vi "Stop Periodic Enqueue Message.vi"(6 "Close Helper Loop (F)":bool, 8 "error in":errorcluster, 11 "Helper Loop":refnum<class "Helper Loop DQMH.lvclass">) -> (0 "error out":errorcluster)   [LabVIEW 2026, in "Helper Loop DQMH.lvclass"]
doc: "周期的処理を終了します。\nClose Helper LoopをTrueにした場合、ヘルパーループを終了し、ユーザーイベントを破棄します。\nClose Helper LoopをFalseにした場合、ヘルパーループを終了させずにヘルパーループを待機状態にします。"
uses:
  Helper Loop DQMH.lvclass
  Helper Loop DQMH.lvclass/Helper Loop DQMH.ctl
  OneDrive/HP/Local/DQMH Helper/Helper Loop/Sub/Helper Loop Map FGV Action.ctl
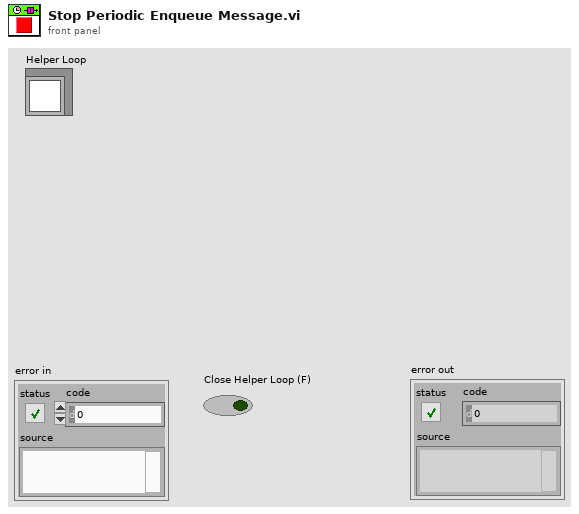
[diagram p1: front panel]
types:
  T1 = typedef "Helper Loop DQMH.lvclass/Helper Loop Map FGV Action.ctl" = enum16{"Get Pausing Helper Loop", "Register Active Helper Loop", "Pause Helper Loop", "Close Helper Loop", "Get All Helper Loops"}
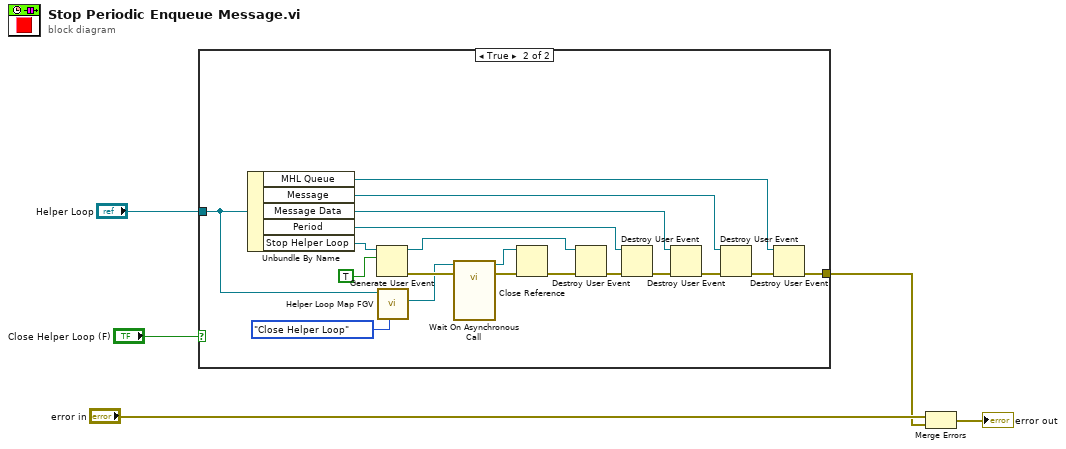
[diagram p0: block diagram]
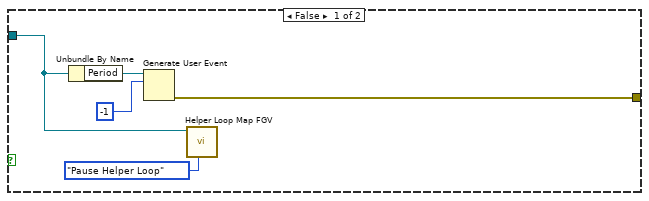
[diagram p2: hidden frame]
diagram:
  n1 = case shown="True" "Close Helper Loop (F)" {
    tunnel: "Helper Loop" -> [w6 w26]
    tunnel: [w8 w18] -> w2
    frame False {
      n2 = Unbundle By Name(w6) -> ("Period"=w10:refnum<user-event>)
      n3 = Generate User Event(user event=w10, event data cluster=-1 ("event data")) -> (error out=w8:errorcluster)  [unwired: 2 in, 1 out]
      n4 = call "Helper Loop Map FGV.vi"("Action"=Helper_Loop_Map_FGV_Action."Pause Helper Loop", "Helper Loop In"=w6) -> ()  [unwired: 6 in, 4 out]
    }
    frame True {
      n5 = Unbundle By Name(w26) -> ("MHL Queue"=w11:refnum<user-event>, "Message"=w12:refnum<user-event>, "Message Data"=w13:refnum<user-event>, "Period"=w14:refnum<user-event>, "Stop Helper Loop"=w29:refnum<user-event>)
      n6 = Generate User Event(user event=w29, event data cluster=TRUE ("event data")) -> (user event out=w20:refnum<user-event>, error out=w27:errorcluster)  [unwired: 2 in]
      n7 = call "Helper Loop Map FGV.vi"("Action"=Helper_Loop_Map_FGV_Action."Close Helper Loop", "Helper Loop In"=w26) -> ("Helper Loop VI Reference Out"=w24:refnum<vi>)  [unwired: 6 in, 3 out]
      n8 = call-by-ref "Wait On Asynchronous Call"(reference=w24, error in=w27) -> (reference out=w22:refnum<vi>, error out=w23:errorcluster)  [unwired: 11 in, 1 out]
      n9 = Close Reference(reference=w22, error in (no error)=w23) -> (error out=w21:errorcluster)
      n10 = Destroy User Event(user event=w20, error in=w21) -> (error out=w17:errorcluster)
      n11 = Destroy User Event(user event=w14, error in=w17) -> (error out=w16:errorcluster)
      n12 = Destroy User Event(user event=w13, error in=w16) -> (error out=w15:errorcluster)
      n13 = Destroy User Event(user event=w12, error in=w15) -> (error out=w19:errorcluster)
      n14 = Destroy User Event(user event=w11, error in=w19) -> (error out=w18:errorcluster)
    }
  }
  n15 = Merge Errors("error in", w2) -> (→"error out":errorcluster)
